vi "Event-TimingDBL.vi"(0 "TimingSec(0.1)":dbl=0.1 format="%#_g秒", 1 "Reset":bool) -> (2 "Timeup":bool)   [LabVIEW 2017]
doc: "<B>#yyll</B>\n秒定时器"
panel:
  # "<B>#yyll</B>\n秒定时器"
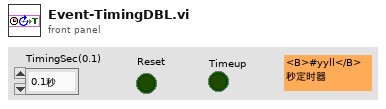
[diagram p1: front panel]
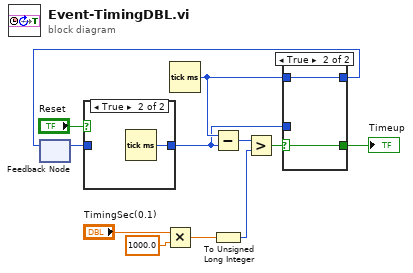
[diagram p0: block diagram]
diagram:
  n1 = feedback #1() -> (w5:u32)  [unwired: 1 in]
  n2 = case shown="True" "Reset" {
    tunnel: w5 -> [w13 _]
    tunnel: [w13 w14] -> w7
    frame False {
    }
    frame True {
      n3 = Tick Count (ms)() -> (millisecond timer value=w14:u32)
    }
  }
  n4 = Multiply(x="TimingSec(0.1)", y=1000.0) -> (x*y=w3:dbl)
  n5 = Tick Count (ms)() -> (millisecond timer value=w10:u32)
  n6 = Subtract(x=w10, y=w7) -> (x-y=w12:u32)
  n7 = To Unsigned Long Integer(number=w3) -> (unsigned 32bit integer=w1:u32)
  n8 = Greater?(x=w12, y=w1) -> (0:w11:bool)
  n9 = case shown="True" w11 {
    selector: w11 -> [_ w16]
    tunnel: w10 -> [_ w17]
    tunnel: [w15 w17] -> w6
    tunnel: [_ w16] -> w9
    tunnel: w7 -> [w15 _]
    frame False {
    }
    frame True {
    }
  }
  "Timeup" <- w9
  n10 = feedback-in #1(w6) -> ()
